vi "VM - Alias Controller.vi"(7 "VC Handle":T1=-1, 8 "error in":errorcluster, 9 "action":u32(ring) items=["nop", "create", "create or rename", "dispose"], 10 "alias":string, 11 "name_spec":string) -> (0 "error out":errorcluster, 2 "dup alias":string, 3 "dup name_spec":string, 5 "dup VC Handle":T1=-1)   [LabVIEW 2021]
doc: "This VI manages the association between a variable and an alias. Refer to the VI help for more details.\n\n<b>VC Handle</b> specifies the handle of the variable context. To operate on a global variable, pass -1 to this input. This input is ignored if the <b>name_spec</b> control refers to a variable by an alias.\n\n<b>name_spec</b> is the name specifier of the desired variable. Usually, it is merely a variable name; however, its generic format is '[name][=alias]', where either 'name' or '=alias' can be omitted but not both.\n\n<b>alias</b> control specifies a new alias associated with the variable.\n\n<b>action</b> control specifies the operation to be performed:\n 'nop' : does nothing.\n 'create' : associates an alias with the variable if it has not been associated yet.\n 'create or rename' : either associates an alias with the variable or renames an alias that is already associated.\n 'dispose' : removes the alias association from the variable.\n\n::: CalcExpress Toolkit :::\nCopyright (c) 2000-2026 Konstantin Shifershteyn. All rights reserved."
uses:
  cetypes.llb/VarMan Variable Context Handle.ctl
  cetypes.llb/VarMan Error Code.ctl
  cersrc/celveng32.dll
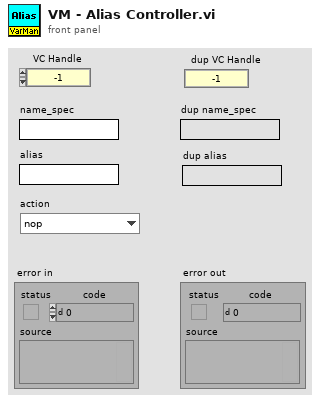
[diagram p1: front panel]
types:
  T1 = typedef "VarMan Variable Context Handle.ctl" = i32
  T2 = typedef "VarMan Error Code.ctl" = u16
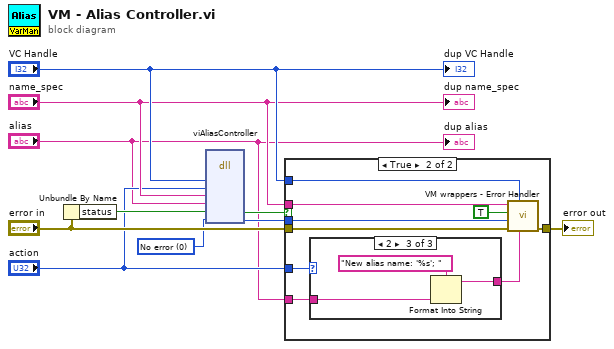
[diagram p0: block diagram]
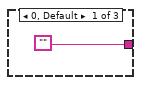
[diagram p3: hidden frame]
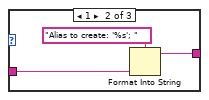
[diagram p4: hidden frame]
diagram:
  w1 = T2 0 items=["No error", "Invalid variable type", "Variable not found", "Variable already exists", "Invalid context handle", "Input error", "Invalid data format", "No history attached", "History already attached", "Invalid history parameters", "Wrong variable name", "Wrong alias name", "Non-unique alias", "Alias not found", "No alias associated", "Alias already associated", "Wrong context name", "Non-unique context name", "Context name not found", "Invalid parameter", "Generic error", "Memory Full", "Unrecognized LV error", "Unknown error code"] ("VarMan error")
  n1 = Unbundle By Name("error in") -> ("status"=w8:bool)
  n2 = dll-call lib="C:/LV Projects/CalcExpress 40 LV2021/vi.lib/addons/CalcExpress/cersrc/celveng*.dll" fn="viAliasController"("vch"="VC Handle", "cmd"="action", "nspec"="name_spec", "alias"="alias", "errf"=w8, "errc"=w1) -> ("errf"=w7:bool, "errc"=w6:T2)  [unwired: 8 in, 2 out]
  n3 = case shown="True" w7 {
    tunnel: "error in" -> [w11 w20]
    tunnel: w6 -> [_ w19]
    tunnel: "name_spec" -> [_ w18]
    tunnel: "VC Handle" -> [_ w17]
    tunnel: [w11 w16] -> w9
    tunnel: "action" -> [_ w14]
    tunnel: "alias" -> [_ w12]
    frame False {
    }
    frame True {
      n4 = case shown="2" w14 {
        tunnel: ["" w23 w26] -> w13
        tunnel: w12 -> [_ w22 w25]
        frame 0, Default {
        }
        frame 1 {
          n5 = Format Into String(format string="Alias to create: '%s'; ", w22) -> (resulting string=w23:string)  [unwired: 2 in, 1 out]
        }
        frame 2 {
          n6 = Format Into String(format string="New alias name: '%s'; ", w25) -> (resulting string=w26:string)  [unwired: 2 in, 1 out]
        }
      }
      n7 = call "VM wrappers - Error Handler.vi"("extra msg"=w13, "VC Handle"=w17, "error before"=w20, "VarMan error"=w19, "show name spec (F)"=TRUE, "name spec"=w18) -> ("error out"=w16:errorcluster)  [unwired: 4 in, 1 out]
    }
  }
  "error out" <- w9
  "dup VC Handle" <- "VC Handle"
  "dup name_spec" <- "name_spec"
  "dup alias" <- "alias"
